vi "Open Pipe (reader).vi"(8 "error in (no error)":errorcluster, 11 "pathname in":string) -> (0 "error out":errorcluster, 3 "pipe reader out":refnum<data-value>)   [LabVIEW 2016, in "Linux RT IPC.Pipes.lvlib" / "Unix Pipe Reader.lvclass"]
doc: "This VI creates a new writer or reader endpoint for accessing the pipe and allowing data transfer."
uses:
  Unix Pipe Reader.lvclass
  C:/Git/SourceTree/LinuxRT-IPC/Source/Pipes/Classes/Unix Pipe/Unix Pipe.lvclass
  C/Controls/file creation flags.ctl
  C/Controls/file status flags.ctl
  C/Controls/epoll operations.ctl
  C/Controls/epoll events.ctl
  Unix Pipe/Unix Pipe.lvclass/Unix Pipe.ctl
  Unix Pipe Reader.lvclass/Unix Pipe Reader.ctl
  C/SubVIs/OR flags U32.vi
  C/SubVIs/error handler.vi
  <vilib>/NI/NI Linux RT Errno/VIs/Public/Get Errno Value for Calling Thread.vi
  C/Linux RT IPC.C.lvlib
  Unix Pipe/Unix Pipe.lvclass
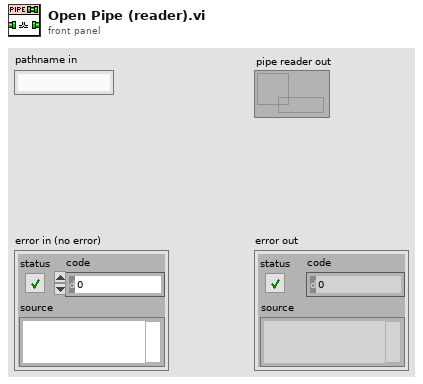
[diagram p1: front panel]
types:
  T1 = typedef "Linux RT IPC.C.lvlib/epoll events.ctl" = u32
  T2 = typedef "Linux RT IPC.C.lvlib/epoll operations.ctl" = u32
  T3 = typedef "Linux RT IPC.C.lvlib/file status flags.ctl" = u32
  T4 = typedef "Linux RT IPC.C.lvlib/file creation flags.ctl" = u32
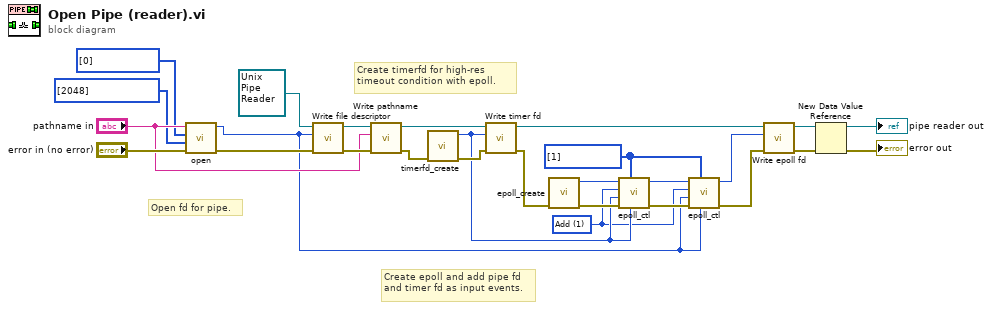
[diagram p0: block diagram]
diagram:
  w9 = T1[] [1] items=["EPOLLIN"=1, "EPOLLPRI"=2, "EPOLLOUT"=4, "EPOLLERR"=8, "EPOLLHUP"=16, "EPOLLRDNORM"=64, "EPOLLRDBAND"=128, "EPOLLWRNORM"=256, "EPOLLWRBAND"=512, "EPOLLMSG"=1024, "EPOLLRDHUP"=8192, "EPOLLWAKEUP"=536870912, "EPOLLONESHOT"=1073741824, "EPOLLET"=2147483648] ("epoll events (default: none)")
  w3 = T2 1 items=["Add"=1, "Delete"=2, "Modify"=3] ("operation")
  w17 = T3[] [2048] items=["O_NONBLOCK"=2048] ("file status flags (default: none)")
  w19 = T4[] [0] items=["O_RDONLY", "O_WRONLY", "O_RDWR"] ("flags")
  # "Create epoll and add pipe fd and timer fd as input events."
  # "Open fd for pipe."
  # "Create timerfd for high-res timeout condition with epoll."
  n1 = call "open.vi"("error in (no error)"="error in (no error)", "file status flags (default: none)"=w17, "file creation flags"=w19, "pathname"="pathname in") -> ("error out"=w24:errorcluster, "file descriptor"=w4:i32)  [unwired: 6 in]
  n2 = call "Write file descriptor.vi"("error in (no error)"=w24, "file descriptor"=w4, "Unix Pipe in"=refnum<class "Unix Pipe Reader.lvclass"> refnum ("Unix Pipes.lvlib:Unix Pipe Reader.lvclass")) -> ("error out"=w22:errorcluster, "Unix Pipe out"=w23:refnum<class "Unix Pipe Reader.lvclass">)  [unwired: 7 in]
  n3 = call "Write pathname.vi"("error in (no error)"=w22, "pathname"="pathname in", "Unix Pipe in"=w23) -> ("error out"=w15:errorcluster, "Unix Pipe out"=w14:refnum<class "Unix Pipe Reader.lvclass">)  [unwired: 7 in]
  n4 = call "timerfd_create.vi"("error in (no error)"=w15) -> ("error out"=w16:errorcluster, "timer fd"=w5:i32)  [unwired: 9 in]
  n5 = call "Write timer fd.vi"("error in (no error)"=w16, "timer fd"=w5, "Unix Pipe Reader in"=w14) -> ("error out"=w13:errorcluster, "Unix Pipe Reader out"=w6:refnum<class "Unix Pipe Reader.lvclass">)  [unwired: 7 in]
  n6 = call "epoll_create.vi"("error in (no error)"=w13) -> ("error out"=w27:errorcluster, "epfd"=w12:i32)  [unwired: 9 in]
  n7 = call "epoll_ctl.vi"("epoll data"=w5, "epoll events (default: none)"=w9, "error in (no error)"=w27, "target fd"=w5, "operation"=w3, "epfd in"=w12) -> ("error out"=w10:errorcluster, "epfd out"=w11:i32)  [unwired: 4 in]
  n8 = call "epoll_ctl.vi"("epoll data"=w4, "epoll events (default: none)"=w9, "error in (no error)"=w10, "target fd"=w4, "operation"=w3, "epfd in"=w11) -> ("error out"=w1:errorcluster, "epfd out"=w2:i32)  [unwired: 4 in]
  n9 = call "Write epoll fd.vi"("error in (no error)"=w1, "epoll fd"=w2, "Unix Pipe Reader in"=w6) -> ("error out"=w7:errorcluster, "Unix Pipe Reader out"=w8:refnum<class "Unix Pipe Reader.lvclass">)  [unwired: 7 in]
  n10 = New Data Value Reference(data value=w8, error in=w7) -> (data value reference=→"pipe reader out":refnum<data-value>, error out=→"error out":errorcluster)
